vi "TEST - File Exists.vi"(8 "error in (no error)":errorcluster) -> (0 "error out":errorcluster, 2 "pass":bool)   [LabVIEW 2020]
uses:
  <userlib>/_OpenG.lib/error/error.llb/openg_error.lvlib
  source/library/openg_file.lvlib
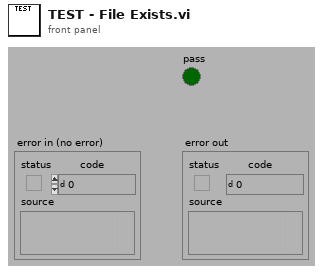
[diagram p1: front panel]
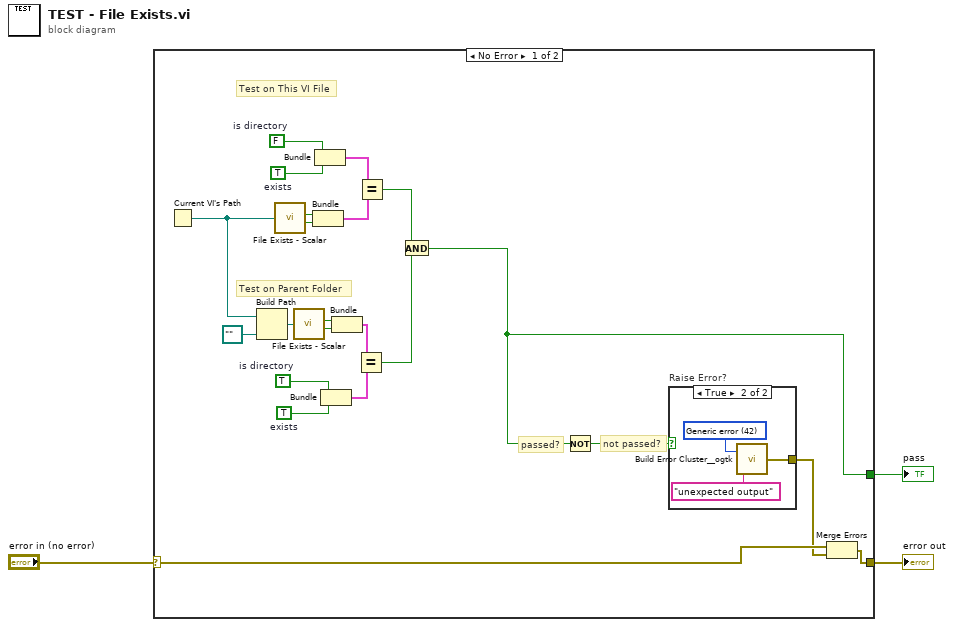
[diagram p0: block diagram]
diagram:
  n1 = case shown="No Error" "error in (no error)" {
    selector: "error in (no error)" -> [w25 w29]
    tunnel: [w4 _] -> w3
    tunnel: [w24 w29] -> w1
    frame No Error {
      w8 = TRUE  # is directory
      w9 = TRUE  # exists
      w20 = TRUE  # exists
      w21 = FALSE  # is directory
      # "Test on This VI File"
      # "Test on Parent Folder"
      # "not passed?"
      # "passed?"
      n2 = Current VI's Path() -> (path=w14:path)
      n3 = Build Path(base path=w14, name or relative path=path ".." ("path")) -> (appended path=w10:path)
      n4 = call "File Exists - Scalar.vi"("file path"=w14) -> ("is directory"=w19:bool, "exists"=w18:bool)  [unwired: 6 in]
      n5 = call "File Exists - Scalar.vi"("file path"=w10) -> ("is directory"=w11:bool, "exists"=w12:bool)  [unwired: 6 in]
      n6 = Bundle("is directory"=w19, "exists"=w18) -> (w16:cluster{"is directory":bool, "exists":bool})  [unwired: 1 in]
      n7 = Bundle("is directory"=w21, "exists"=w20) -> (w17:cluster{"is directory":bool, "exists":bool})  [unwired: 1 in]
      n8 = Bundle("is directory"=w8, "exists"=w9) -> (w7:cluster{"is directory":bool, "exists":bool})  [unwired: 1 in]
      n9 = Bundle("is directory"=w11, "exists"=w12) -> (w6:cluster{"is directory":bool, "exists":bool})  [unwired: 1 in]
      n10 = Equal?(x=w6, y=w7) -> (x = y?=w5:bool)
      n11 = Equal?(x=w17, y=w16) -> (x = y?=w15:bool)
      n12 = And(x=w15, y=w5) -> (x .and. y?=w4:bool)
      n13 = Not(x=w4) -> (.not. x?=w22:bool)
      n14 = case "Raise Error?" shown="True" w22 {
        tunnel: [_ w26] -> w23
        frame False {
        }
        frame True {
          w27 = 42 items=["No error", "Argument error", "Memory is full", "Out of zone", "End of file", "File already open", "Generic file I/O error", "File not found", "File permission error", "Disk is full", "Duplicate path", "Too many files open", "System feature not enabled", "Resource file not found", "Cannot add resource", "Resource not found", "Image not found", "Image memory error", "Pen does not exist", "Config type invalid", "Config token not found", "Config parse error", "Config memory error", "Bad external code format", "Bad external code offset", "External code not present", "Null window", "Destroy window error", "Null menu", "Print aborted", "Bad print record", "Print driver error", "Windows error during printing", "Memory error during printing", "Print dialog error", "Generic print error", "Invalid device refnum", "Device not found", "Device parameter error", "Device unit error", "Cannot open device", "Device call aborted", "Generic error", "Cancelled by user", "Object ID too low", "Object ID too high", "Object not in heap", "Unknown heap", "Unknown object (invalid DefProc)", "Unknown object (DefProc not in table)", "Message out of range", "Invalid (null) method", "Unknown message", "Manager call not supported", "Bad address", "Network operation in progress", "Network operation timed out", "Connection is busy", "Network attribute not supported", "Network error", "Address in use", "System out of memory", "Connection aborted", "Connection refused", "Not connected", "Already connected", "Connection closed", "Initialization error (interapplication manager)", "Bad occurrence", "Wait on unbound occurrence handler", "Occurrence queue overflow", "Datalog type conflict", "Unused", "Unrecognized type (interapplication manager)", "Memory corrupt", "Failed to make temporary DLL", "Old CIN version", "Drag socket not found", "Failed to load drop-object", "Failed to register OLE object", "Failed to release OLE object", "Format specifier type mismatch", "Unknown format specifier", "Too few format specifiers", "Too many format specifiers", "Scan failed", "Newer CIN version", "Error converting to variant", "Runtime menu error", "Password tampered", "Variant attribute not found", "Incompatible variant data type", "Event data is not available", "Event Store is not present", "Occurrence is not found", "Event Queue is not created", "Event info is not available", "Refnum passed is NULL", "Error retrieving Class GUID", "Error retrieving CoClass GUID", "Error retrieving TypeLib GUID.", "Bad built application magic bytes.", "Specific driver is different from the specific driver associated with the Logical Name.", "There is no session opened to the class driver.", "Max Error", "MAX - Error with config objects", "MAX - Error loading configuration", "MAX - Group not supported"]
          n15 = call <userlib>:"Build Error Cluster__ogtk.vi"("String to Prepend to source (\"\")"="unexpected output" ("String to Prepend to source (\"\")"), "code"=w27) -> ("error out"=w26:errorcluster)
        }
      }
      n16 = Merge Errors(w25, w23) -> (w24:errorcluster)
    }
    frame Error {
    }
  }
  "pass" <- w3
  "error out" <- w1
